vi "GraphViz Generator UI Wrapper.vi"(10 "Modules Configurations":refnum<class "TBM module configuration.lvclass">[](array[class]), 11 "engine configuration in":refnum<class "engine configuration.lvclass">) -> ()   [LabVIEW 2014, in "GraphViz Mapping Visualizer.lvlib"]
uses:
  GraphViz Mapping Visualizer.lvlib
  <vilib>/NI/Module Execution Interface/Engine Configuration/engine configuration.lvclass
  <vilib>/NI/Tag Bus Module Framework/module configuration/TBM module configuration.lvclass
  System.Windows.Forms
  <vilib>/event_ctls.llb/sizeaction.ctl
  System.Drawing
  Configuration Editor/Classes/Engine Mappings/Engine Mappings.lvclass
panel:
  in  "Tab Control":enum32{"Setup", "Image"}(tab)
  in  "Modules to View":T1(array[cluster])
  in  "Supported Colors":string[](array[string])=["dodgerblue", "cadetblue1", "darkgoldenrod1", "gainsboro", "palegreen", "peachpuff", "violet", "skyblue", "yellow", "seagreen1", "tomato", "thistle", "slateblue1", "orange", "palevioletred1"]
  in  "Show Unmapped Channels":bool=TRUE
  in  "Show Tag Labels":bool
  in  "Zoom":bool=TRUE
  in  "Generate":bool
  in  "PictureBox":refnum<k24>(container)
  # "Generation Options"
  # "Supported colors list found at \nhttp://www.graphviz.org/doc/info/colors.html"
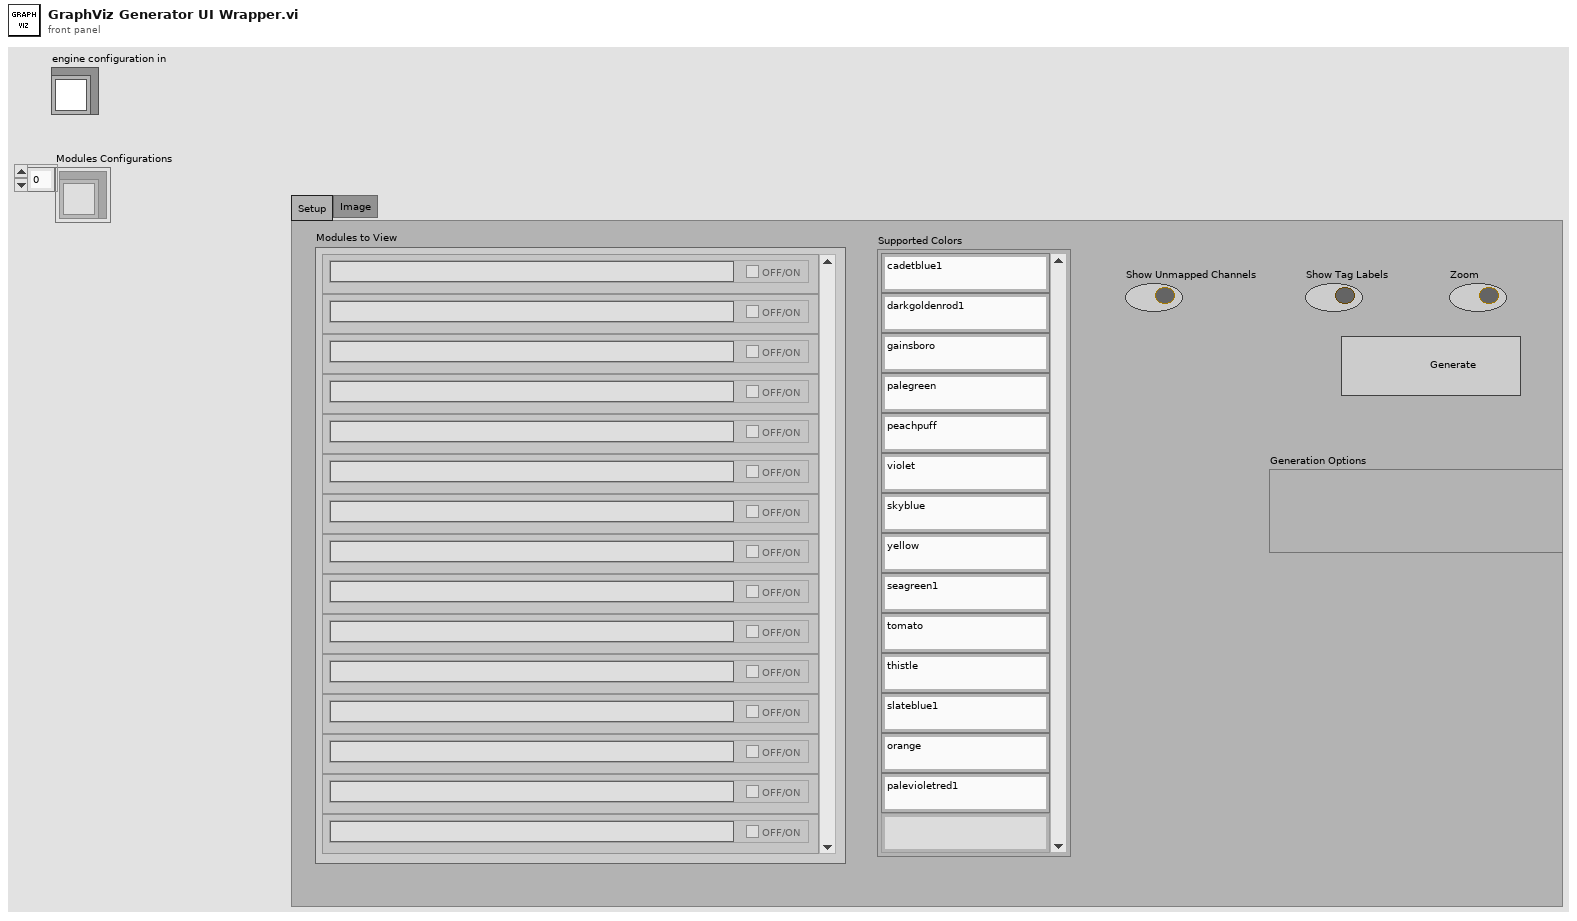
[diagram p1: front panel]
types:
  T1 = cluster{"Module Display Name":string, "View?":bool}[]
  T2 = typedef "PL Framework Configuration Tool.lvlib/Engine Mappings.lvclass/module information.ctl" = cluster{"display name":string, "instance id":string, "channels":refnum<class "TBM channel.lvclass">[]}
  T3 = cluster{"Module Display Name":string, "View?":bool}
  T4 = enum16{"open", "replace", "create", "open or create", "replace or create", "replace or create with confirmation"}
  T5 = typedef "sizeaction.ctl" = enum32{"Minimized", "Maximized", "Resized"}
  T6 = typedef "panelstate.ctl" = enum32{"Standard", "Minimized", "Maximized"}
  T7 = typedef "LVRectTypeDef.ctl" = cluster{"Left":i16, "Top":i16, "Right":i16, "Bottom":i16}
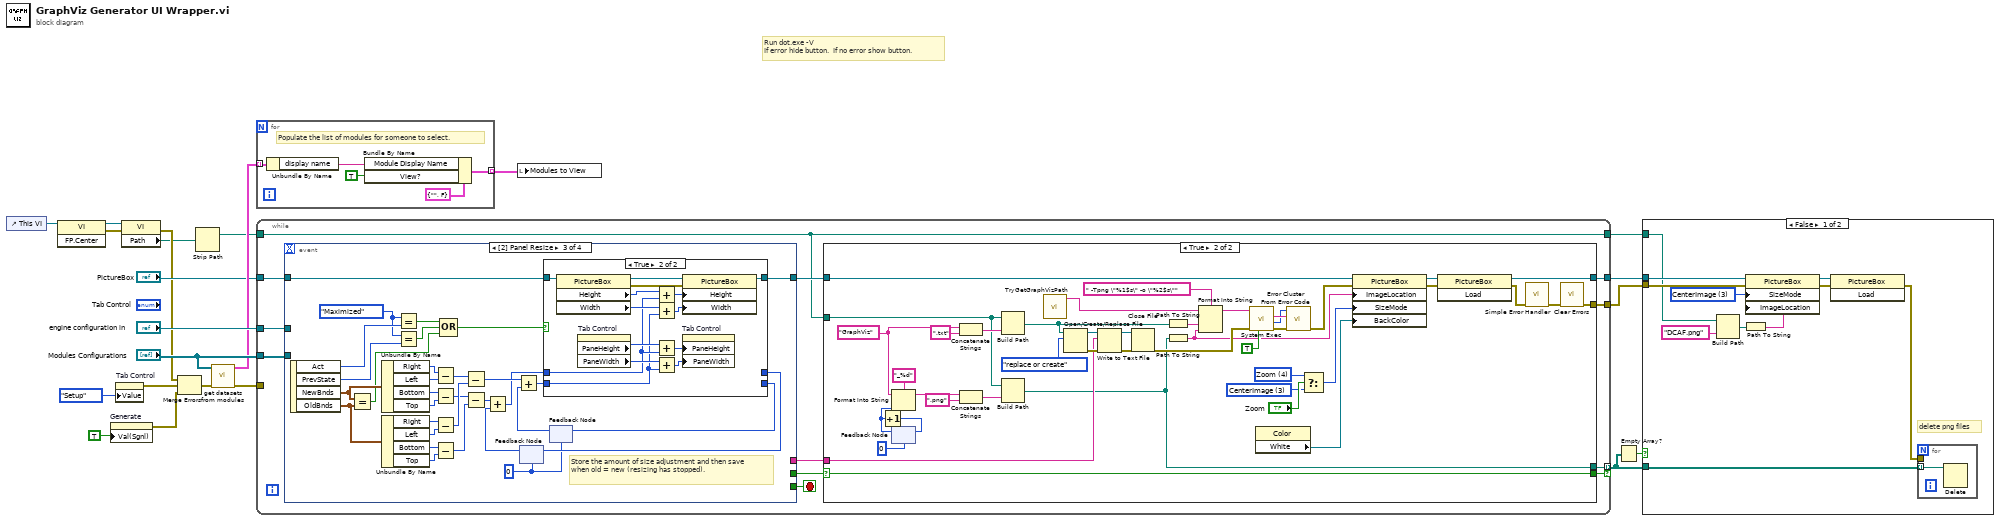
[diagram p0: block diagram]
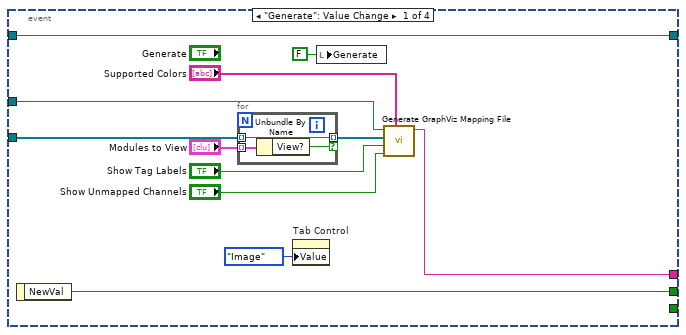
[diagram p4: hidden frame]
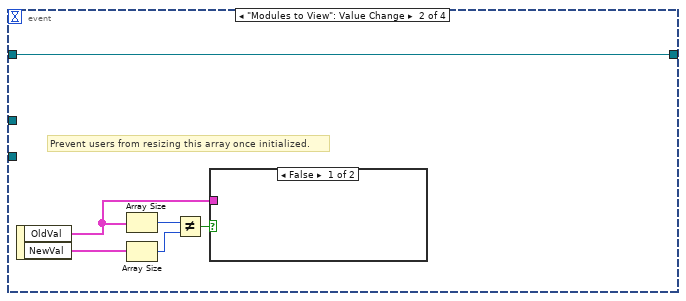
[diagram p5: hidden frame]
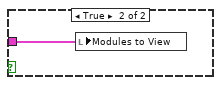
[diagram p6: hidden frame]
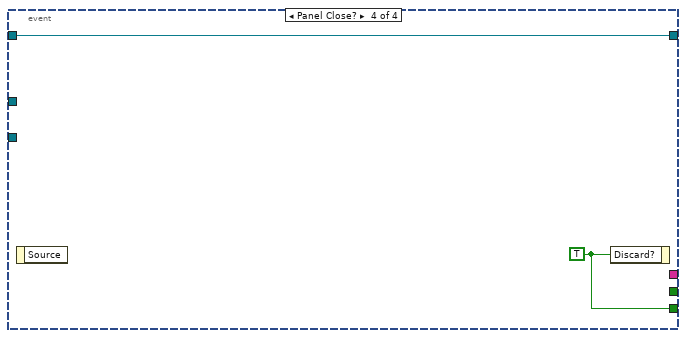
[diagram p8: hidden frame]
diagram:
  # "Run dot.exe -V\nIf error hide button.  If no error show button."
  n1 = control-ref of="This VI"() -> (w16:refnum<vi>)
  n2 = invoke class="VI" method="FP.Center"(reference=w16) -> (reference out=w4:refnum<vi>, error out=w6:errorcluster)  [unwired: 2 in, 1 out]
  n3 = property on="Generate" class="Bool (strict)"("Val(Sgnl)"=TRUE) -> (error out=w9:errorcluster)  [unwired: 2 in, 1 out]
  n4 = property on="Tab Control" class="TabCtl (strict)"("Value"=enum32{"Setup", "Image", "Text"}."Setup" ("Tab Control")) -> (error out=w10:errorcluster)  [unwired: 2 in, 1 out]
  n5 = property class="VI"(reference=w4, error in=w6) -> (error out=w5:errorcluster, "Path"=w2:path)  [unwired: 1 out]
  n6 = Merge Errors(w5, w10, w9) -> (w8:errorcluster)
  n7 = Strip Path(path=w2) -> (stripped path=w1:path)  [unwired: 1 out]
  n8 = call "get datasets from modules.vi"("error in"=w8, "Modules Configurations"="Modules Configurations") -> ("error out"=w7:errorcluster, "module datasets"=w20:T2[])  [unwired: 8 in]
  n9 = for {
    tunnel: w20 -> [w27] mode=indexing
    tunnel: [w23] -> w19 mode=indexing
    # "Populate the list of modules for someone to select."
    n10 = Unbundle By Name(w27) -> ("display name"=w24:string)
    n11 = Bundle By Name(cluster=T3 {"Module Display Name"="", "View?"=FALSE} ("Cluster"), "Module Display Name"=w24, "View?"=TRUE) -> (w23:T3)
  }
  n12 = while {
    tunnel: "engine configuration in" -> [w39]
    tunnel: "Modules Configurations" -> [w38]
    tunnel: [w34] -> w12 mode=indexing if=w33
    tunnel: [w30] -> w13
    tunnel: "PictureBox" -> [w32]
    tunnel: [w31] -> w14
    tunnel: w7 -> [_]
    tunnel: w1 -> [w28]
    tunnel: [w28] -> w3
    stop <- w37 stop-if-true
    n13 = event shown="[2] Panel Resize" {
      selector: _ -> [_ _ _ _]
      dyn-events: _ -> [_ _ _ _]
      timeout: _ -> [_ _ _ _]
      tunnel: w39 -> [w91 _ _ _]
      tunnel: w38 -> [w90 _ _ _]
      tunnel: [_ _ _ w156] -> w37
      tunnel: [w85 _ _ _] -> w36
      tunnel: [w92 _ _ _] -> w35
      tunnel: w32 -> [w84 w99 w109 w155]
      tunnel: [w84 w99 w106 w155] -> w29
      event "Generate": Value Change {
        n14 = event-data() -> ("NewVal"=w85:bool)  [unwired: 1 in]
        n15 = for {
          tunnel: "Modules to View" -> [w98] mode=indexing
          tunnel: w90 -> [w97] mode=indexing
          tunnel: [w97] -> w89 mode=indexing if=w96
          n16 = Unbundle By Name(w98) -> ("View?"=w96:bool)
        }
        n17 = property on="Tab Control" class="TabCtl (strict)"("Value"=enum32{"Setup", "Image", "Text"}."Image" ("Tab Control")) -> ()  [unwired: 2 in, 2 out]
        n18 = local write "Generate"(FALSE ("Generate")) -> ()
        n19 = call "Generate GraphViz Mapping File.vi"("supported colors"="Supported Colors", "Show Unmapped Channels?"="Show Unmapped Channels", "Show Tag Labels?"="Show Tag Labels", "Modules Configurations"=w89, "engine configuration in"=w91) -> ("output to graphviz"=w92:string)  [unwired: 6 in]
      }
      event "Modules to View": Value Change {
        # "Prevent users from resizing this array once initialized."
        n20 = event-data() -> ("OldVal"=w100:T1, "NewVal"=w104:T1)  [unwired: 1 in]
        n21 = Array Size(array=w100) -> (size(s)=w103:i32)
        n22 = Array Size(array=w104) -> (size(s)=w102:i32)
        n23 = Not Equal?(x=w103, y=w102) -> (x != y?=w101:bool)
        n24 = case shown="False" w101 {
          tunnel: w100 -> [_ w105]
          frame False {
          }
          frame True {
            n25 = local write "Modules to View"(w105) -> ()
          }
        }
      }
      event Panel Resize {
        w112 = sizeaction."Maximized" ("Act")
        w110 = 0 ("x+y")
        # "Store the amount of size adjustment and then save when old = new (resizing has stopped)."
        n26 = event-data() -> ("Act"=w115:T5, "PrevState"=w114:T6, "NewBnds"=w113:T7, "OldBnds"=w107:T7)  [unwired: 1 in]
        n27 = Equal?(x=w113, y=w107) -> (x = y?=w108:bool)
        n28 = Unbundle By Name(w113) -> ("Right"=w123:i16, "Left"=w122:i16, "Bottom"=w121:i16, "Top"=w120:i16)
        n29 = Unbundle By Name(w107) -> ("Right"=w126:i16, "Left"=w127:i16, "Bottom"=w125:i16, "Top"=w124:i16)
        n30 = Equal?(x=w112, y=w115) -> (x = y?=w130:bool)
        n31 = Equal?(x=w112, y=w114) -> (x = y?=w129:bool)
        n32 = Subtract(x=w123, y=w122) -> (x-y=w119:i16)
        n33 = Subtract(x=w121, y=w120) -> (x-y=w117:i16)
        n34 = Subtract(x=w126, y=w127) -> (x-y=w118:i16)
        n35 = Subtract(x=w125, y=w124) -> (x-y=w116:i16)
        n36 = Compound Arithmetic op=OR(w130, w129, w108) -> (w128:bool)
        n37 = Subtract(x=w119, y=w118) -> (x-y=w136:i16)
        n38 = Subtract(x=w117, y=w116) -> (x-y=w137:i16)
        n39 = feedback #1(w110) -> (w133:i32)
        n40 = Add(x=w137, y=w133) -> (x+y=w135:i32)
        n41 = feedback #2(w110) -> (w111:i32)
        n42 = Add(x=w136, y=w111) -> (x+y=w134:i32)
        n43 = case shown="True" w128 {
          tunnel: w109 -> [w138 w148]
          tunnel: w135 -> [w140 w143]
          tunnel: w134 -> [w139 w142]
          tunnel: [w140 _] -> w132
          tunnel: [w139 _] -> w131
          tunnel: [w138 w141] -> w106
          frame False {
          }
          frame True {
            n44 = property class="PictureBox"(reference=w148) -> (reference out=w154:refnum<k24>, error out=w149:errorcluster, "Height"=w153:i32, "Width"=w152:i32)  [unwired: 1 in]
            n45 = property on="Tab Control" class="TabCtl (strict)"() -> ("PaneHeight"=w147:u32, "PaneWidth"=w145:u32)  [unwired: 2 in, 2 out]
            n46 = Add(x=w153, y=w143) -> (x+y=w151:i32)
            n47 = Add(x=w152, y=w142) -> (x+y=w150:i32)
            n48 = Add(x=w147, y=w143) -> (x+y=w146:u32)
            n49 = Add(x=w145, y=w142) -> (x+y=w144:u32)
            n50 = property class="PictureBox"(reference=w154, error in=w149, "Height"=w151, "Width"=w150) -> (reference out=w141:refnum<k24>)  [unwired: 1 out]
            n51 = property on="Tab Control" class="TabCtl (strict)"("PaneHeight"=w146, "PaneWidth"=w144) -> ()  [unwired: 2 in, 2 out]
          }
        }
        n52 = feedback-in #1(w132) -> ()
        n53 = feedback-in #2(w131) -> ()
      }
      event Panel Close? {
        w156 = TRUE ("Discard?")
        n54 = event-data() -> ()  [unwired: 1 in, 1 out]
        n55 = event-data("Discard?"=w156) -> ()  [unwired: 1 in, 1 out]
      }
    }
    n56 = case shown="True" w36 {
      selector: w36 -> [_ w67]
      tunnel: w35 -> [_ w62]
      tunnel: [_ w43] -> w34
      tunnel: [_ w67] -> w33
      tunnel: w29 -> [w40 w49]
      tunnel: [w40 w47] -> w31
      tunnel: [_ w44] -> w30
      tunnel: w28 -> [_ w42]
      frame False {
      }
      frame True {
        w70 = 4 items=["Normal", "StretchImage", "AutoSize", "CenterImage", "Zoom"] ("SizeMode")
        w69 = 3 items=["Normal", "StretchImage", "AutoSize", "CenterImage", "Zoom"] ("SizeMode")
        w58 = "GraphViz" ("name or relative path")
        n57 = feedback #3(0) -> (w56:i32)
        n58 = Increment(x=w56) -> (x+1=w55:i32)
        n59 = Format Into String(format string="_%d", initial string=w58, w56) -> (resulting string=w60:string)  [unwired: 1 in, 1 out]
        n60 = feedback-in #3(w55) -> ()
        n61 = Concatenate Strings(w58, ".txt" ("name or relative path")) -> (w57:string)
        n62 = Concatenate Strings(w60, ".png" ("string")) -> (w73:string)
        n63 = Build Path(base path=w42, name or relative path=w57) -> (appended path=w78:path)
        n64 = Build Path(base path=w42, name or relative path=w73) -> (appended path=w43:path)
        n65 = call "TryGetGraphVizPath.vi"() -> ("Path"=w41:string)  [unwired: 10 in, 1 out]
        n66 = Open/Create/Replace File(file path (use dialog)=w78, operation (0:open)=T4."replace or create") -> (refnum out=w83:refnum<file>, error out=w82:errorcluster)  [unwired: 4 in, 1 out]
        n67 = Write to Text File(file (use dialog)=w83, text=w62, error in=w82) -> (refnum out=w80:refnum<file>, error out=w81:errorcluster)  [unwired: 1 in, 1 out]
        n68 = Close File(refnum=w80, error in=w81) -> (error out=w79:errorcluster)  [unwired: 1 out]
        n69 = Path To String(path=w78) -> (string=w51:string)
        n70 = Path To String(path=w43) -> (string=w48:string)
        n71 = Format Into String(format string=" -Tpng \"%1$s\" -o \"%2$s\"" ("name or relative path"), initial string=w41, w51, w48) -> (resulting string=w50:string)  [unwired: 1 in, 1 out]
        n72 = call <vilib>:"System Exec.vi"("run minimized? (F)"=TRUE, "error in (no error)"=w79, "command line"=w50) -> ("error out"=w66:errorcluster, "return code"=w64:i32, "standard error"=w65:string)  [unwired: 5 in, 1 out]
        n73 = property class="Color"() -> ("White"=w72:refnum<k24>)  [unwired: 2 in, 2 out]
        n74 = call <vilib>:"Error Cluster From Error Code.vi"("error in (no error)"=w66, "error message (\"\")"=w65, "error code (0)"=w64) -> ("error out"=w63:errorcluster)  [unwired: 6 in]
        n75 = Select(t=w70, s="Zoom", f=w69) -> (s? t:f=w68:i32)
        n76 = property class="PictureBox"(reference=w49, error in=w63, "ImageLocation"=w48, "SizeMode"=w68, "BackColor"=w72) -> (reference out=w76:refnum<k24>, error out=w75:errorcluster)
        n77 = invoke class="PictureBox" method="Load"(reference=w76, error in=w75) -> (reference out=w47:refnum<k24>, error out=w45:errorcluster)  [unwired: 1 in, 1 out]
        n78 = call <vilib>:"Simple Error Handler.vi"("error in (no error)"=w45) -> ("error out"=w46:errorcluster)  [unwired: 4 in, 4 out]
        n79 = call <vilib>:"Clear Errors.vi"("error in (no error)"=w46) -> ("error out"=w44:errorcluster)  [unwired: 5 in, 1 out]
      }
    }
  }
  n80 = local write "Modules to View"(w19) -> ()
  n81 = Empty Array?(array=w12) -> (empty?=w11:bool)
  n82 = case shown="False" w11 {
    tunnel: w14 -> [w167 _]
    tunnel: w13 -> [w166 _]
    tunnel: w12 -> [w163 _]
    tunnel: w3 -> [w157 _]
    frame False {
      w161 = 3 items=["Normal", "StretchImage", "AutoSize", "CenterImage", "Zoom"] ("SizeMode")
      # "delete png files"
      n83 = Build Path(base path=w157, name or relative path="DCAF.png") -> (appended path=w160:path)
      n84 = Path To String(path=w160) -> (string=w159:string)
      n85 = property class="PictureBox"(reference=w167, error in=w166, "SizeMode"=w161, "ImageLocation"=w159) -> (reference out=w165:refnum<k24>, error out=w164:errorcluster)
      n86 = invoke class="PictureBox" method="Load"(reference=w165, error in=w164) -> (error out=w158:errorcluster)  [unwired: 1 in, 2 out]
      n87 = for {
        tunnel: w163 -> [w168] mode=indexing
        tunnel: w158 -> [_]
        n88 = Delete(path (use dialog)=w168) -> ()  [unwired: 4 in, 3 out]
      }
    }
    frame True {
    }
  }
